vi "Add Text.vi"(8 "error in":errorcluster, 10 "text":string, 11 "ToastBuilder in":refnum<class "ToastBuilder.lvclass">) -> (0 "error out":errorcluster, 3 "ToastBuilder out":refnum<class "ToastBuilder.lvclass">)   [LabVIEW 2026, in "ToastNotification.lvlib" / "ToastBuilder.lvclass"]
doc: "Append a text block to the native toast builder. The displayed text is not automatically returned as an activation argument. Call before Show. Skip on incoming error and preserve the input builder. Copies of the class share the same native builder."
uses:
  ToastBuilder.lvclass
  ToastBuilder.lvclass/ToastBuilder.ctl
  Read Builder Reference.vi
  Write Builder Reference.vi
  Toast Native/Toast Native.lvlib
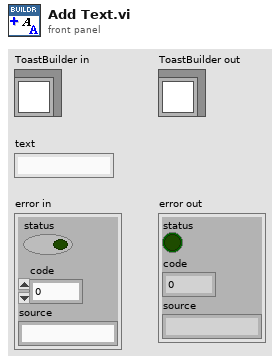
[diagram p1: front panel]
types:
  T1 = typedef "ToastNotification.lvlib/ToastBuilder.lvclass/Builder Reference.ctl" = refnum<k24>
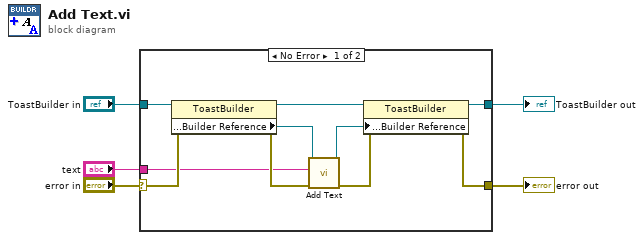
[diagram p0: block diagram]
diagram:
  n1 = case shown="No Error" "error in" {
    selector: "error in" -> [w13 w16]
    tunnel: "ToastBuilder in" -> [w15 w17]
    tunnel: [w12 w17] -> w3
    tunnel: [w11 w16] -> w2
    tunnel: "text" -> [w6 _]
    frame No Error {
      n2 = property class="ToastBuilder"(reference=w15, error in=w13) -> (reference out=w14:refnum<class "ToastBuilder.lvclass">, error out=w8:errorcluster, "Public:Properties:Builder Reference"=w10:T1)
      n3 = call "Add Text.vi"("error in (no error)"=w8, "text"=w6, "reference"=w10) -> ("error out"=w7:errorcluster, "reference out"=w9:refnum<k24>)  [unwired: 7 in]
      n4 = property class="ToastBuilder"(reference=w14, error in=w7, "Public:Properties:Builder Reference"=w9) -> (reference out=w12:refnum<class "ToastBuilder.lvclass">, error out=w11:errorcluster)
    }
    frame Error {
    }
  }
  "ToastBuilder out" <- w3
  "error out" <- w2
